vi "FT10xx系列_Parameter_sample_1.0.3.vi"() -> ()   [LabVIEW 2017]
uses:
  National Instruments/LabVIEW 2017/user.lib/smncsftmt/smncsftmt.lvlib
panel:
  in  "停止按钮":bool
  out "START 计数率":u32
  out "error out":errorcluster
  in  "阻抗抗S":i32(ring) items=["50Ω"=1, "1MΩ"=0]
  in  "触发":i32(ring) items=["上升沿", "下降沿"]
  in  "阈值电平(mv)":i32=-100 min=-2000 max=3000 step=1 format="%.0fmV"
  out "已连接？":bool
  out "CH8 计数率":u32
  out "CH7 计数率":u32
  out "CH6 计数率":u32
  out "CH5 计数率":u32
  out "CH4 计数率":u32
  out "CH3 计数率":u32
  out "CH2 计数率":u32
  out "CH1 计数率":u32
  in  "阈值电平(mv) 8":i32=-100 min=-2000 max=3000 step=1 format="%.0fmV"
  in  "阻抗抗8":i32(ring) items=["50Ω"=1, "1MΩ"=0]
  in  "触发  8":i32(ring) items=["上升沿", "下降沿"]
  in  "阈值电平(mv) 7":i32=-100 min=-2000 max=3000 step=1 format="%.0fmV"
  in  "阻抗抗7":i32(ring) items=["50Ω"=1, "1MΩ"=0]
  in  "触发  7":i32(ring) items=["上升沿", "下降沿"]
  in  "阈值电平(mv) 6":i32=-100 min=-2000 max=3000 step=1 format="%.0fmV"
  in  "阻抗抗6":i32(ring) items=["50Ω"=1, "1MΩ"=0]
  in  "触发  6":i32(ring) items=["上升沿", "下降沿"]
  in  "阈值电平(mv) 5":i32=-100 min=-2000 max=3000 step=1 format="%.0fmV"
  in  "阻抗抗5":i32(ring) items=["50Ω"=1, "1MΩ"=0]
  in  "触发  5":i32(ring) items=["上升沿", "下降沿"]
  in  "阈值电平(mv) 4":i32=-100 min=-2000 max=3000 step=1 format="%.0fmV"
  in  "阻抗抗4":i32(ring) items=["50Ω"=1, "1MΩ"=0]
  in  "触发  4":i32(ring) items=["上升沿", "下降沿"]
  in  "阈值电平(mv) 3":i32=-100 min=-2000 max=3000 step=1 format="%.0fmV"
  in  "阻抗抗3":i32(ring) items=["50Ω"=1, "1MΩ"=0]
  in  "触发  3":i32(ring) items=["上升沿", "下降沿"]
  in  "阈值电平(mv) 2":i32=-100 min=-2000 max=3000 step=1 format="%.0fmV"
  in  "阻抗抗2":i32(ring) items=["50Ω"=1, "1MΩ"=0]
  in  "触发  2":i32(ring) items=["上升沿", "下降沿"]
  in  "阈值电平(mv) 1":i32=-100 min=-2000 max=3000 step=1 format="%.0fmV"
  in  "阻抗":i32(ring) items=["50Ω"=1, "1MΩ"=0]
  in  "触发  1":i32(ring) items=["上升沿", "下降沿"]
  # "FT10XX系列参数设置"
  # "参数设置"
  # "计数显示"
  # "同步信号（START)"
  # "测量通道STOP(1-8)"
  # "1"
  # "2"
  # "3"
  # "4"
  # "5"
  # "6"
  # "7"
  # "8"
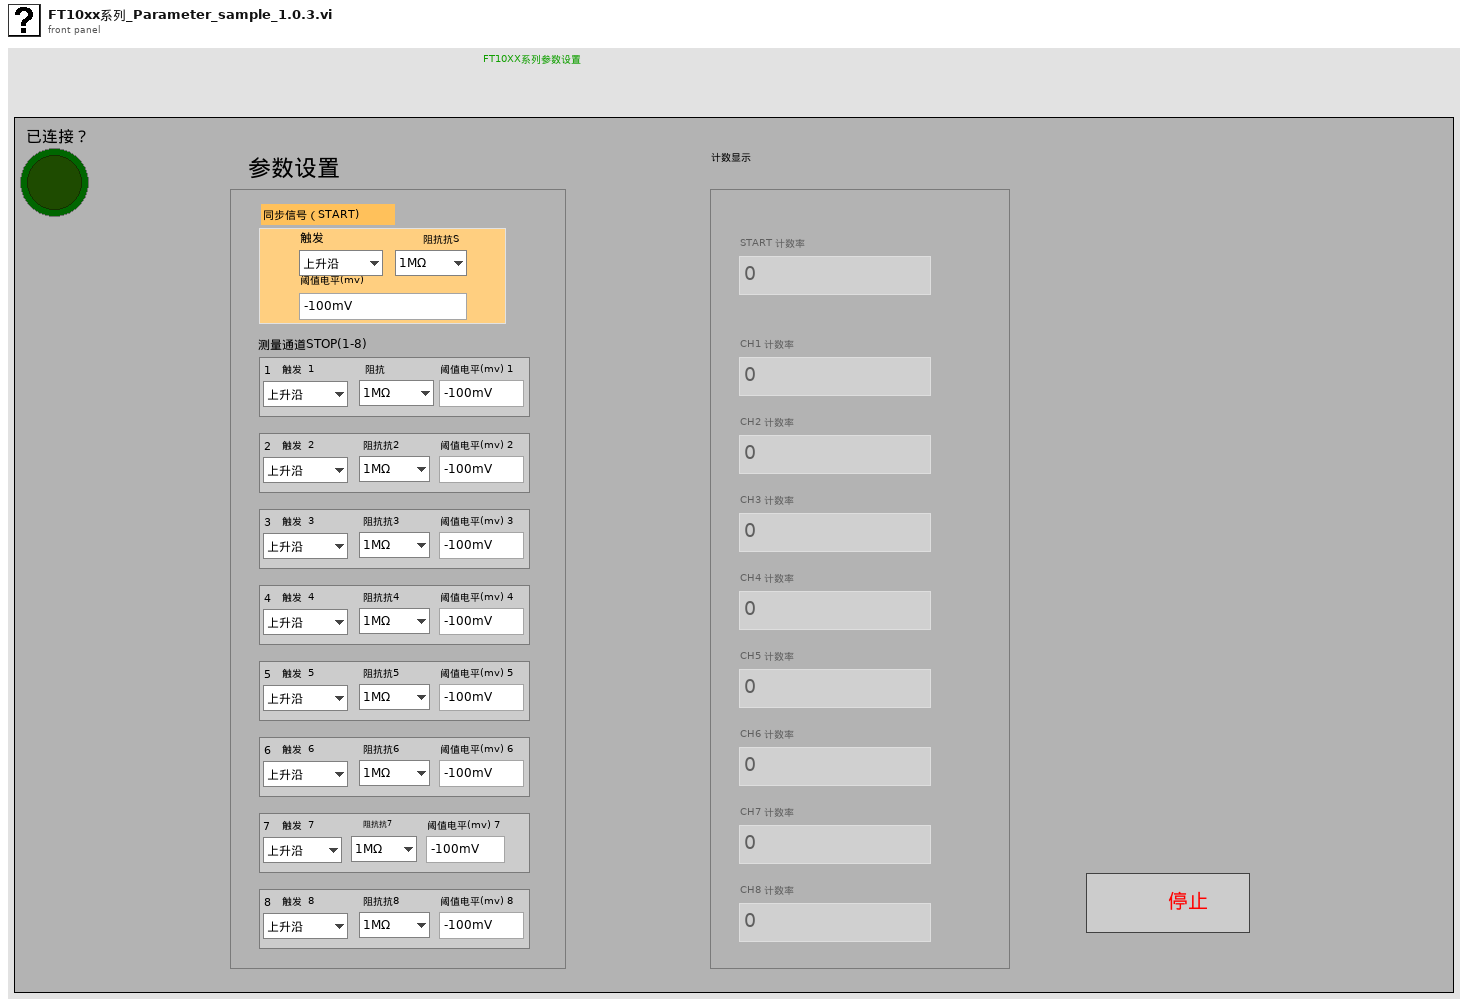
[diagram p1: front panel]
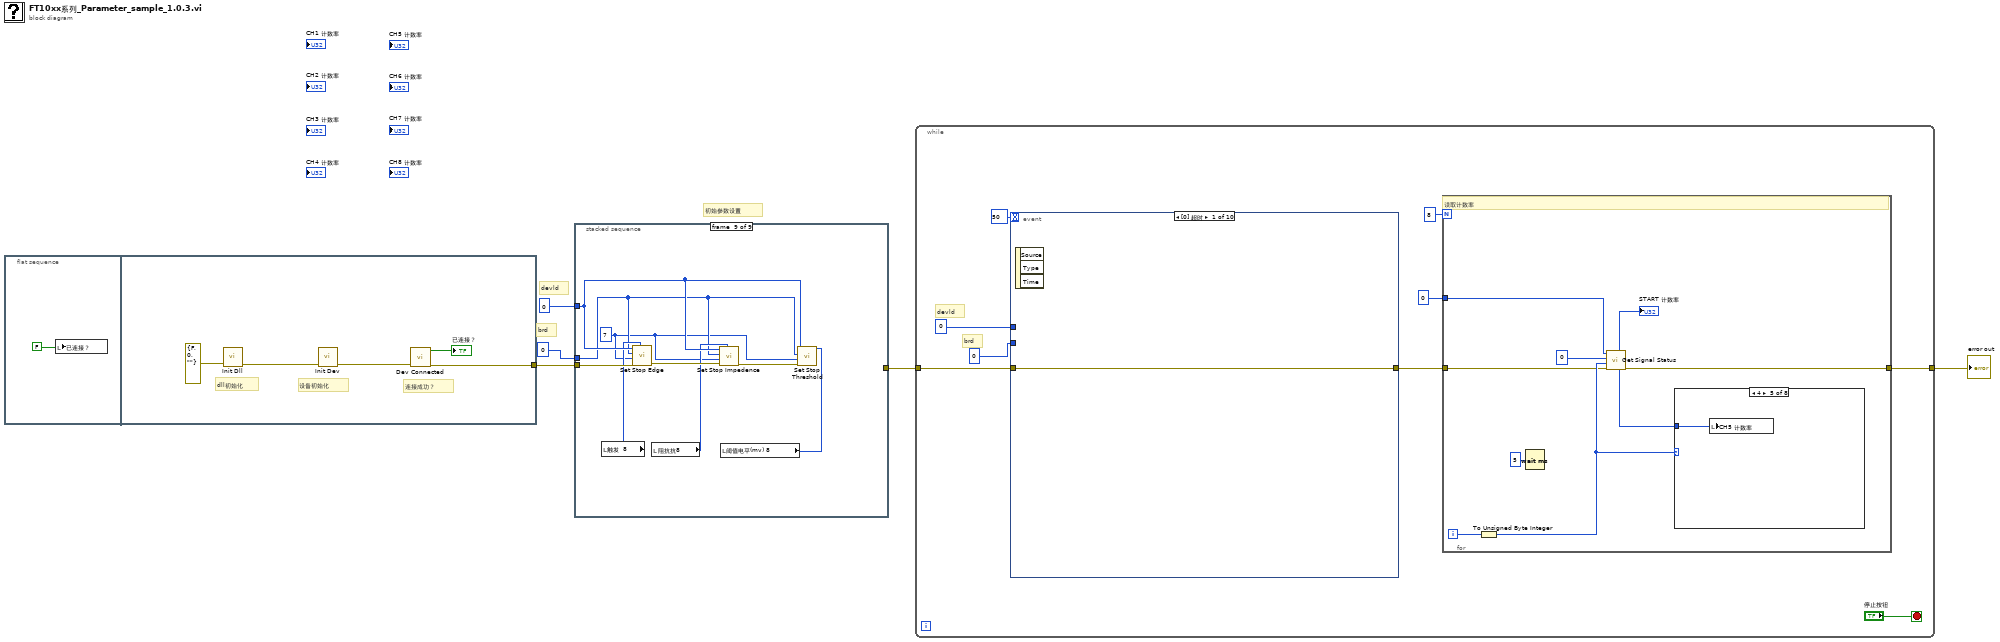
[diagram p0: block diagram]
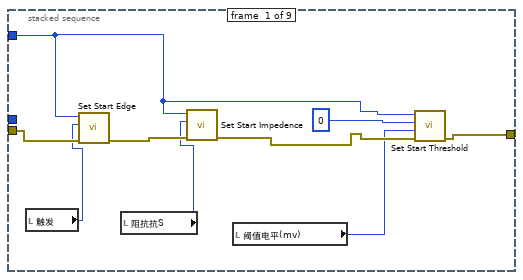
[diagram p2: hidden frame]
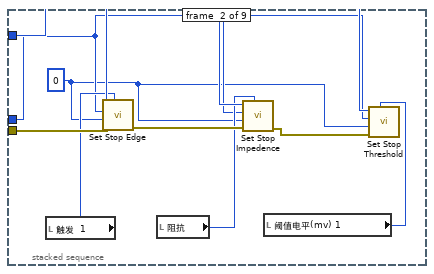
[diagram p3: hidden frame]
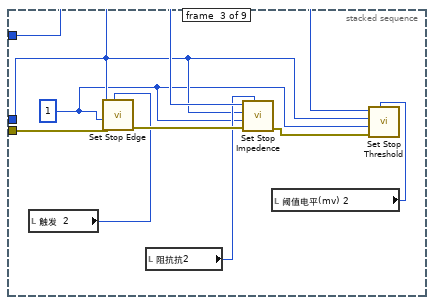
[diagram p4: hidden frame]
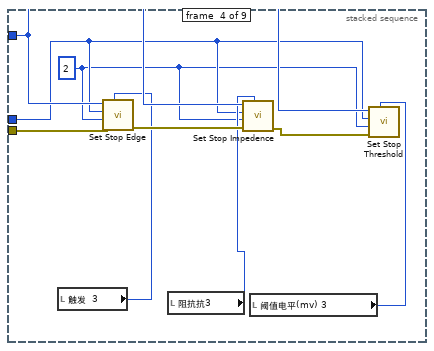
[diagram p5: hidden frame]
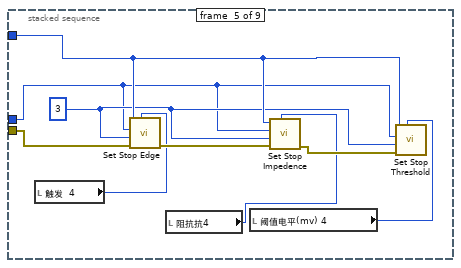
[diagram p6: hidden frame]
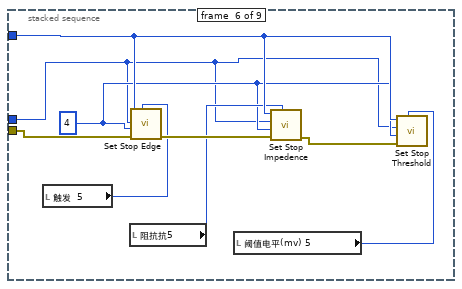
[diagram p7: hidden frame]
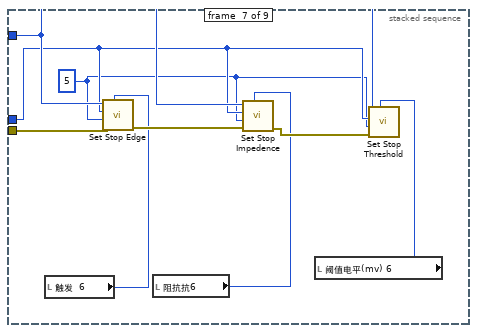
[diagram p8: hidden frame]
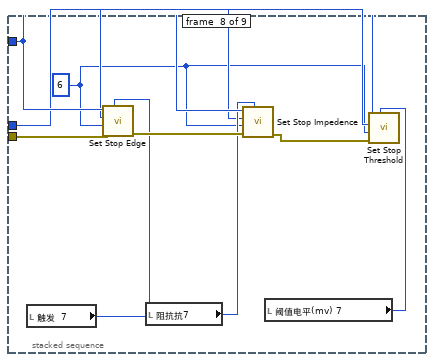
[diagram p9: hidden frame]
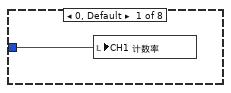
[diagram p10: hidden frame]
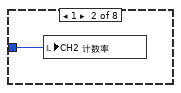
[diagram p11: hidden frame]
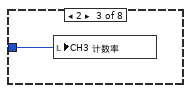
[diagram p12: hidden frame]
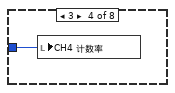
[diagram p13: hidden frame]
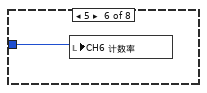
[diagram p14: hidden frame]
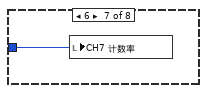
[diagram p15: hidden frame]
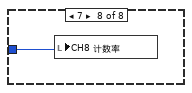
[diagram p16: hidden frame]
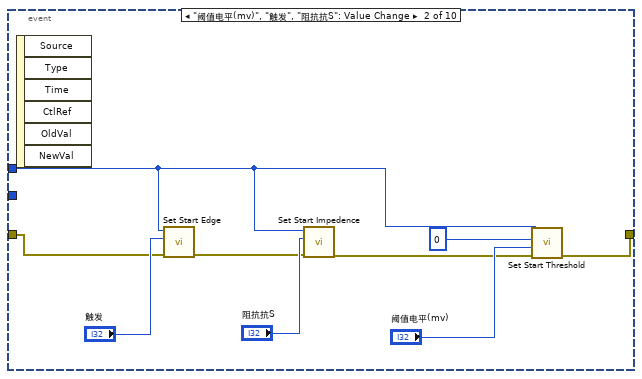
[diagram p17: hidden frame]
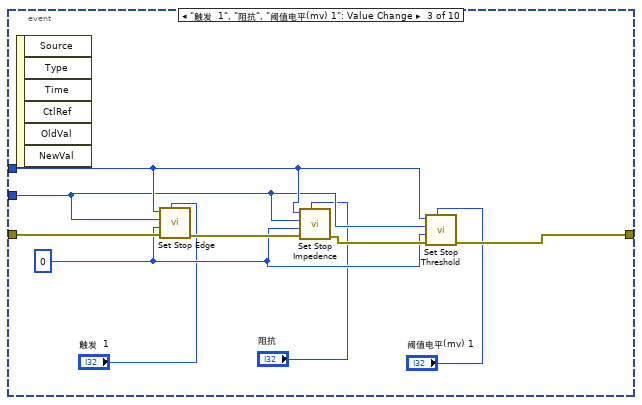
[diagram p18: hidden frame]
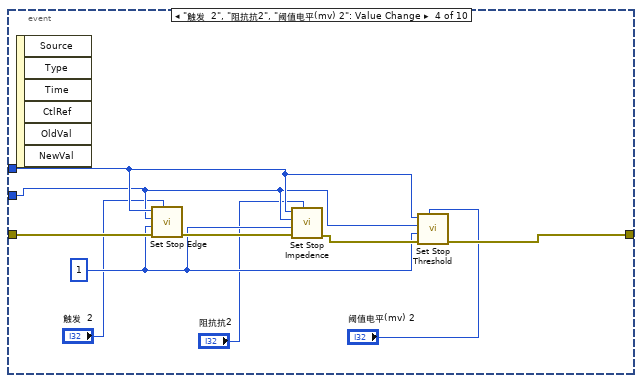
[diagram p19: hidden frame]
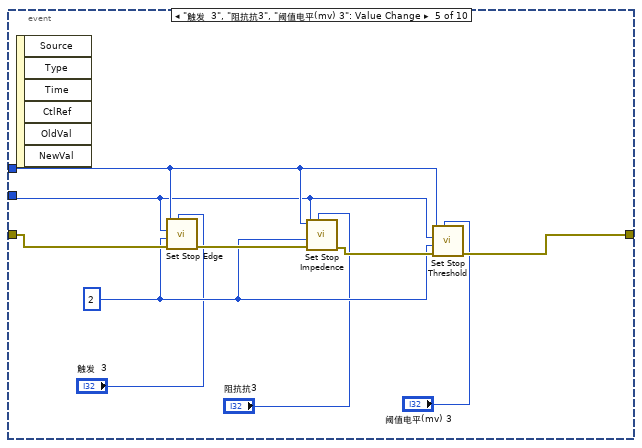
[diagram p20: hidden frame]
diagram:
  # "初始参数设置"
  # "brd"
  # "devld"
  n1 = flat-sequence {
    tunnel: [w8] -> w3
    frame #0 {
      n2 = local write "已连接？"(FALSE) -> ()
    }
    frame #1 {
      # "连接成功？"
      # "设备初始化"
      # "dll初始化"
      n3 = call "Init Dll.vi"("error in (no error)"=errorcluster {"status"=FALSE, "code"=0, "source"=""}) -> ("error out"=w11:errorcluster)  [unwired: 9 in, 1 out]
      n4 = call "Init Dev.vi"("error in (no error)"=w11) -> ("error out"=w10:errorcluster)  [unwired: 9 in, 1 out]
      n5 = call "Dev Connected.vi"("error in (no error)"=w10) -> ("error out"=w8:errorcluster, "function return"=→"已连接？":bool)  [unwired: 9 in]
    }
  }
  n6 = stacked-sequence {
    tunnel: w3 -> [w17 w28 w37 w46 w56 w65 w73 w82 w91]
    tunnel: 0 -> [w16 w29 w38 w47 w53 w62 w74 w83 w92]
    tunnel: [w12 _ _ _ _ _ _ _ _] -> w4
    tunnel: 0 -> [_ w22 w31 w40 w48 w57 w67 w76 w85]
    frame #0 {
      n7 = local read "触发"() -> (w15:i32)
      n8 = call "Set Start Edge.vi"("error in (no error)"=w17, "nEdge"=w15, "nDevId"=w16) -> ("error out"=w18:errorcluster)  [unwired: 7 in, 1 out]
      n9 = local read "阻抗抗S"() -> (w14:i32)
      n10 = call "Set Start Impedence.vi"("error in (no error)"=w18, "nImpedence"=w14, "nDevId"=w16) -> ("error out"=w20:errorcluster)  [unwired: 7 in, 1 out]
      n11 = local read "阈值电平(mv)"() -> (w13:i32)
      n12 = call "Set Start Threshold.vi"("error in (no error)"=w20, "nStartThrsh"=w13, "nBoard"=0 ("startThrsh"), "nDevId"=w16) -> ("error out"=w12:errorcluster)  [unwired: 6 in, 1 out]
    }
    frame #1 {
      w21 = 0
      n13 = local read "触发  1"() -> (w24:i32)
      n14 = call "Set Stop Edge.vi"("nEdge"=w24, "error in (no error)"=w28, "nChannel"=w21, "nBoard"=w22, "nDevId"=w29) -> ("error out"=w27:errorcluster)  [unwired: 5 in, 1 out]
      n15 = local read "阻抗"() -> (w23:i32)
      n16 = call "Set Stop Impedence.vi"("nImpedence"=w23, "error in (no error)"=w27, "nChannel"=w21, "nBoard"=w22, "nDevId"=w29) -> ("error out"=w26:errorcluster)  [unwired: 5 in, 1 out]
      n17 = local read "阈值电平(mv) 1"() -> (w25:i32)
      n18 = call "Set Stop Threshold.vi"("nStopThrsh"=w25, "error in (no error)"=w26, "nChannel"=w21, "nBoard"=w22, "nDevId"=w29) -> ()  [unwired: 5 in, 2 out]
    }
    frame #2 {
      w30 = 1
      n19 = local read "触发  2"() -> (w34:i32)
      n20 = call "Set Stop Edge.vi"("nEdge"=w34, "error in (no error)"=w37, "nChannel"=w30, "nBoard"=w31, "nDevId"=w38) -> ("error out"=w36:errorcluster)  [unwired: 5 in, 1 out]
      n21 = local read "阻抗抗2"() -> (w33:i32)
      n22 = call "Set Stop Impedence.vi"("nImpedence"=w33, "error in (no error)"=w36, "nChannel"=w30, "nBoard"=w31, "nDevId"=w38) -> ("error out"=w35:errorcluster)  [unwired: 5 in, 1 out]
      n23 = local read "阈值电平(mv) 2"() -> (w32:i32)
      n24 = call "Set Stop Threshold.vi"("nStopThrsh"=w32, "error in (no error)"=w35, "nChannel"=w30, "nBoard"=w31, "nDevId"=w38) -> ()  [unwired: 5 in, 2 out]
    }
    frame #3 {
      w39 = 2
      n25 = local read "触发  3"() -> (w43:i32)
      n26 = call "Set Stop Edge.vi"("nEdge"=w43, "error in (no error)"=w46, "nChannel"=w39, "nBoard"=w40, "nDevId"=w47) -> ("error out"=w45:errorcluster)  [unwired: 5 in, 1 out]
      n27 = local read "阻抗抗3"() -> (w42:i32)
      n28 = call "Set Stop Impedence.vi"("nImpedence"=w42, "error in (no error)"=w45, "nChannel"=w39, "nBoard"=w40, "nDevId"=w47) -> ("error out"=w44:errorcluster)  [unwired: 5 in, 1 out]
      n29 = local read "阈值电平(mv) 3"() -> (w41:i32)
      n30 = call "Set Stop Threshold.vi"("nStopThrsh"=w41, "error in (no error)"=w44, "nChannel"=w39, "nBoard"=w40, "nDevId"=w47) -> ()  [unwired: 5 in, 2 out]
    }
    frame #4 {
      w49 = 3
      n31 = local read "触发  4"() -> (w50:i32)
      n32 = call "Set Stop Edge.vi"("nEdge"=w50, "error in (no error)"=w56, "nChannel"=w49, "nBoard"=w48, "nDevId"=w53) -> ("error out"=w55:errorcluster)  [unwired: 5 in, 1 out]
      n33 = local read "阻抗抗4"() -> (w51:i32)
      n34 = local read "阈值电平(mv) 4"() -> (w52:i32)
      n35 = call "Set Stop Impedence.vi"("nImpedence"=w51, "error in (no error)"=w55, "nChannel"=w49, "nBoard"=w48, "nDevId"=w53) -> ("error out"=w54:errorcluster)  [unwired: 5 in, 1 out]
      n36 = call "Set Stop Threshold.vi"("nStopThrsh"=w52, "error in (no error)"=w54, "nChannel"=w49, "nBoard"=w48, "nDevId"=w53) -> ()  [unwired: 5 in, 2 out]
    }
    frame #5 {
      w58 = 4
      n37 = local read "触发  5"() -> (w61:i32)
      n38 = local read "阻抗抗5"() -> (w60:i32)
      n39 = call "Set Stop Edge.vi"("nEdge"=w61, "error in (no error)"=w65, "nChannel"=w58, "nBoard"=w57, "nDevId"=w62) -> ("error out"=w64:errorcluster)  [unwired: 5 in, 1 out]
      n40 = local read "阈值电平(mv) 5"() -> (w59:i32)
      n41 = call "Set Stop Impedence.vi"("nImpedence"=w60, "error in (no error)"=w64, "nChannel"=w58, "nBoard"=w57, "nDevId"=w62) -> ("error out"=w63:errorcluster)  [unwired: 5 in, 1 out]
      n42 = call "Set Stop Threshold.vi"("nStopThrsh"=w59, "error in (no error)"=w63, "nChannel"=w58, "nBoard"=w57, "nDevId"=w62) -> ()  [unwired: 5 in, 2 out]
    }
    frame #6 {
      w66 = 5
      n43 = local read "触发  6"() -> (w68:i32)
      n44 = call "Set Stop Edge.vi"("nEdge"=w68, "error in (no error)"=w73, "nChannel"=w66, "nBoard"=w67, "nDevId"=w74) -> ("error out"=w72:errorcluster)  [unwired: 5 in, 1 out]
      n45 = local read "阻抗抗6"() -> (w69:i32)
      n46 = call "Set Stop Impedence.vi"("nImpedence"=w69, "error in (no error)"=w72, "nChannel"=w66, "nBoard"=w67, "nDevId"=w74) -> ("error out"=w71:errorcluster)  [unwired: 5 in, 1 out]
      n47 = local read "阈值电平(mv) 6"() -> (w70:i32)
      n48 = call "Set Stop Threshold.vi"("nStopThrsh"=w70, "error in (no error)"=w71, "nChannel"=w66, "nBoard"=w67, "nDevId"=w74) -> ()  [unwired: 5 in, 2 out]
    }
    frame #7 {
      w75 = 6
      n49 = local read "触发  7"() -> (w77:i32)
      n50 = call "Set Stop Edge.vi"("nEdge"=w77, "error in (no error)"=w82, "nChannel"=w75, "nBoard"=w76, "nDevId"=w83) -> ("error out"=w81:errorcluster)  [unwired: 5 in, 1 out]
      n51 = local read "阻抗抗7"() -> (w78:i32)
      n52 = call "Set Stop Impedence.vi"("nImpedence"=w78, "error in (no error)"=w81, "nChannel"=w75, "nBoard"=w76, "nDevId"=w83) -> ("error out"=w80:errorcluster)  [unwired: 5 in, 1 out]
      n53 = local read "阈值电平(mv) 7"() -> (w79:i32)
      n54 = call "Set Stop Threshold.vi"("nStopThrsh"=w79, "error in (no error)"=w80, "nChannel"=w75, "nBoard"=w76, "nDevId"=w83) -> ()  [unwired: 5 in, 2 out]
    }
    frame #8 {
      w84 = 7
      n55 = local read "触发  8"() -> (w88:i32)
      n56 = call "Set Stop Edge.vi"("nEdge"=w88, "error in (no error)"=w91, "nChannel"=w84, "nBoard"=w85, "nDevId"=w92) -> ("error out"=w90:errorcluster)  [unwired: 5 in, 1 out]
      n57 = local read "阻抗抗8"() -> (w87:i32)
      n58 = call "Set Stop Impedence.vi"("nImpedence"=w87, "error in (no error)"=w90, "nChannel"=w84, "nBoard"=w85, "nDevId"=w92) -> ("error out"=w89:errorcluster)  [unwired: 5 in, 1 out]
      n59 = local read "阈值电平(mv) 8"() -> (w86:i32)
      n60 = call "Set Stop Threshold.vi"("nStopThrsh"=w86, "error in (no error)"=w89, "nChannel"=w84, "nBoard"=w85, "nDevId"=w92) -> ()  [unwired: 5 in, 2 out]
    }
  }
  n61 = while {
    tunnel: w4 -> [w97]
    tunnel: [w95] -> w2
    stop <- "停止按钮" stop-if-true
    # "brd"
    # "devld"
    n62 = event shown="[0] 超时" {
      selector: _ -> [_ _ _ _ _ _ _ _ _ _]
      dyn-events: _ -> [_ _ _ _ _ _ _ _ _ _]
      timeout: 50 -> [_ _ _ _ _ _ _ _ _ _]
      tunnel: 0 -> [_ w125 w134 w144 w154 w164 w174 w184 w194 w204]
      tunnel: [w119 w120 w135 w145 w155 w165 w175 w185 w195 w205] -> w96
      tunnel: w97 -> [w119 w121 w138 w148 w158 w168 w178 w188 w198 w208]
      tunnel: 0 -> [_ _ w133 w143 w153 w162 w169 w183 w193 w203]
      event Timeout {
        n63 = event-data() -> ()  [unwired: 1 in, 3 out]
      }
      event "阈值电平(mv)", "触发", "阻抗抗S": Value Change {
        n64 = event-data() -> ()  [unwired: 1 in, 6 out]
        n65 = call "Set Start Edge.vi"("error in (no error)"=w121, "nEdge"="触发", "nDevId"=w125) -> ("error out"=w126:errorcluster)  [unwired: 7 in, 1 out]
        n66 = call "Set Start Impedence.vi"("error in (no error)"=w126, "nImpedence"="阻抗抗S", "nDevId"=w125) -> ("error out"=w122:errorcluster)  [unwired: 7 in, 1 out]
        n67 = call "Set Start Threshold.vi"("error in (no error)"=w122, "nStartThrsh"="阈值电平(mv)", "nBoard"=0 ("startThrsh"), "nDevId"=w125) -> ("error out"=w120:errorcluster)  [unwired: 6 in, 1 out]
      }
      event "触发  1", "阻抗", "阈值电平(mv) 1": Value Change {
        w132 = 0
        n68 = event-data() -> ()  [unwired: 1 in, 6 out]
        n69 = call "Set Stop Edge.vi"("nEdge"="触发  1", "error in (no error)"=w138, "nChannel"=w132, "nBoard"=w133, "nDevId"=w134) -> ("error out"=w137:errorcluster)  [unwired: 5 in, 1 out]
        n70 = call "Set Stop Impedence.vi"("nImpedence"="阻抗", "error in (no error)"=w137, "nChannel"=w132, "nBoard"=w133, "nDevId"=w134) -> ("error out"=w136:errorcluster)  [unwired: 5 in, 1 out]
        n71 = call "Set Stop Threshold.vi"("nStopThrsh"="阈值电平(mv) 1", "error in (no error)"=w136, "nChannel"=w132, "nBoard"=w133, "nDevId"=w134) -> ("error out"=w135:errorcluster)  [unwired: 5 in, 1 out]
      }
      event "触发  2", "阻抗抗2", "阈值电平(mv) 2": Value Change {
        w142 = 1
        n72 = event-data() -> ()  [unwired: 1 in, 6 out]
        n73 = call "Set Stop Edge.vi"("nEdge"="触发  2", "error in (no error)"=w148, "nChannel"=w142, "nBoard"=w143, "nDevId"=w144) -> ("error out"=w147:errorcluster)  [unwired: 5 in, 1 out]
        n74 = call "Set Stop Impedence.vi"("nImpedence"="阻抗抗2", "error in (no error)"=w147, "nChannel"=w142, "nBoard"=w143, "nDevId"=w144) -> ("error out"=w146:errorcluster)  [unwired: 5 in, 1 out]
        n75 = call "Set Stop Threshold.vi"("nStopThrsh"="阈值电平(mv) 2", "error in (no error)"=w146, "nChannel"=w142, "nBoard"=w143, "nDevId"=w144) -> ("error out"=w145:errorcluster)  [unwired: 5 in, 1 out]
      }
      event "触发  3", "阻抗抗3", "阈值电平(mv) 3": Value Change {
        w152 = 2
        n76 = event-data() -> ()  [unwired: 1 in, 6 out]
        n77 = call "Set Stop Edge.vi"("nEdge"="触发  3", "error in (no error)"=w158, "nChannel"=w152, "nBoard"=w153, "nDevId"=w154) -> ("error out"=w157:errorcluster)  [unwired: 5 in, 1 out]
        n78 = call "Set Stop Impedence.vi"("nImpedence"="阻抗抗3", "error in (no error)"=w157, "nChannel"=w152, "nBoard"=w153, "nDevId"=w154) -> ("error out"=w156:errorcluster)  [unwired: 5 in, 1 out]
        n79 = call "Set Stop Threshold.vi"("nStopThrsh"="阈值电平(mv) 3", "error in (no error)"=w156, "nChannel"=w152, "nBoard"=w153, "nDevId"=w154) -> ("error out"=w155:errorcluster)  [unwired: 5 in, 1 out]
      }
      event "触发  4", "阻抗抗4", "阈值电平(mv) 4": Value Change {
        w163 = 3
        n80 = event-data() -> ()  [unwired: 1 in, 6 out]
        n81 = call "Set Stop Edge.vi"("nEdge"="触发  4", "error in (no error)"=w168, "nChannel"=w163, "nBoard"=w162, "nDevId"=w164) -> ("error out"=w167:errorcluster)  [unwired: 5 in, 1 out]
        n82 = call "Set Stop Impedence.vi"("nImpedence"="阻抗抗4", "error in (no error)"=w167, "nChannel"=w163, "nBoard"=w162, "nDevId"=w164) -> ("error out"=w166:errorcluster)  [unwired: 5 in, 1 out]
        n83 = call "Set Stop Threshold.vi"("nStopThrsh"="阈值电平(mv) 4", "error in (no error)"=w166, "nChannel"=w163, "nBoard"=w162, "nDevId"=w164) -> ("error out"=w165:errorcluster)  [unwired: 5 in, 1 out]
      }
      event "触发  5", "阻抗抗5", "阈值电平(mv) 5": Value Change {
        w170 = 4
        n84 = event-data() -> ()  [unwired: 1 in, 6 out]
        n85 = call "Set Stop Edge.vi"("nEdge"="触发  5", "error in (no error)"=w178, "nChannel"=w170, "nBoard"=w169, "nDevId"=w174) -> ("error out"=w177:errorcluster)  [unwired: 5 in, 1 out]
        n86 = call "Set Stop Impedence.vi"("nImpedence"="阻抗抗5", "error in (no error)"=w177, "nChannel"=w170, "nBoard"=w169, "nDevId"=w174) -> ("error out"=w176:errorcluster)  [unwired: 5 in, 1 out]
        n87 = call "Set Stop Threshold.vi"("nStopThrsh"="阈值电平(mv) 5", "error in (no error)"=w176, "nChannel"=w170, "nBoard"=w169, "nDevId"=w174) -> ("error out"=w175:errorcluster)  [unwired: 5 in, 1 out]
      }
      event "触发  6", "阻抗抗6", "阈值电平(mv) 6": Value Change {
        w182 = 5
        n88 = event-data() -> ()  [unwired: 1 in, 6 out]
        n89 = call "Set Stop Edge.vi"("nEdge"="触发  6", "error in (no error)"=w188, "nChannel"=w182, "nBoard"=w183, "nDevId"=w184) -> ("error out"=w187:errorcluster)  [unwired: 5 in, 1 out]
        n90 = call "Set Stop Impedence.vi"("nImpedence"="阻抗抗6", "error in (no error)"=w187, "nChannel"=w182, "nBoard"=w183, "nDevId"=w184) -> ("error out"=w186:errorcluster)  [unwired: 5 in, 1 out]
        n91 = call "Set Stop Threshold.vi"("nStopThrsh"="阈值电平(mv) 6", "error in (no error)"=w186, "nChannel"=w182, "nBoard"=w183, "nDevId"=w184) -> ("error out"=w185:errorcluster)  [unwired: 5 in, 1 out]
      }
      event "触发  7", "阻抗抗7", "阈值电平(mv) 7": Value Change {
        w192 = 6
        n92 = event-data() -> ()  [unwired: 1 in, 6 out]
        n93 = call "Set Stop Edge.vi"("nEdge"="触发  7", "error in (no error)"=w198, "nChannel"=w192, "nBoard"=w193, "nDevId"=w194) -> ("error out"=w197:errorcluster)  [unwired: 5 in, 1 out]
        n94 = call "Set Stop Impedence.vi"("nImpedence"="阻抗抗7", "error in (no error)"=w197, "nChannel"=w192, "nBoard"=w193, "nDevId"=w194) -> ("error out"=w196:errorcluster)  [unwired: 5 in, 1 out]
        n95 = call "Set Stop Threshold.vi"("nStopThrsh"="阈值电平(mv) 7", "error in (no error)"=w196, "nChannel"=w192, "nBoard"=w193, "nDevId"=w194) -> ("error out"=w195:errorcluster)  [unwired: 5 in, 1 out]
      }
      event "触发  8", "阻抗抗8", "阈值电平(mv) 8": Value Change {
        w199 = 7
        n96 = event-data() -> ()  [unwired: 1 in, 6 out]
        n97 = call "Set Stop Edge.vi"("nEdge"="触发  8", "error in (no error)"=w208, "nChannel"=w199, "nBoard"=w203, "nDevId"=w204) -> ("error out"=w207:errorcluster)  [unwired: 5 in, 1 out]
        n98 = call "Set Stop Impedence.vi"("nImpedence"="阻抗抗8", "error in (no error)"=w207, "nChannel"=w199, "nBoard"=w203, "nDevId"=w204) -> ("error out"=w206:errorcluster)  [unwired: 5 in, 1 out]
        n99 = call "Set Stop Threshold.vi"("nStopThrsh"="阈值电平(mv) 8", "error in (no error)"=w206, "nChannel"=w199, "nBoard"=w203, "nDevId"=w204) -> ("error out"=w205:errorcluster)  [unwired: 5 in, 1 out]
      }
    }
    n100 = for {
      N: 8 -> [_]
      tunnel: 0 -> [w109]
      tunnel: w96 -> [w105]
      tunnel: [w104] -> w95
      i -> [w110]
      # "读取计数率"
      n101 = To Unsigned Byte Integer(number=w110) -> (unsigned 8bit integer=w107:u8)
      n102 = Wait (ms)(milliseconds to wait=u32 5 ("等待时间（毫秒）")) -> ()  [unwired: 1 out]
      n103 = call "Get Signal Status.vi"("error in (no error)"=w105, "nChannel"=w107, "nBoard"=0, "nDevId"=w109) -> ("error out"=w104:errorcluster, "ptrStopCount out"=w106:u32, "ptrStartCount out"=→"START 计数率":u32)  [unwired: 4 in, 1 out]
      n104 = case shown="4" w107 {
        tunnel: w106 -> [w111 w112 w113 w114 w115 w116 w117 w118]
        frame 0, Default {
          n105 = local write "CH1 计数率"(w111) -> ()
        }
        frame 1 {
          n106 = local write "CH2 计数率"(w112) -> ()
        }
        frame 2 {
          n107 = local write "CH3 计数率"(w113) -> ()
        }
        frame 3 {
          n108 = local write "CH4 计数率"(w114) -> ()
        }
        frame 4 {
          n109 = local write "CH5 计数率"(w115) -> ()
        }
        frame 5 {
          n110 = local write "CH6 计数率"(w116) -> ()
        }
        frame 6 {
          n111 = local write "CH7 计数率"(w117) -> ()
        }
        frame 7 {
          n112 = local write "CH8 计数率"(w118) -> ()
        }
      }
    }
  }
  "error out" <- w2
